vi "Save Library.vi"(8 "error in (no error)":errorcluster, 10 "Save Path (empty)":path, 11 "Library in":refnum<vi>) -> (0 "error out":errorcluster, 3 "Library out":refnum<vi>)   [LabVIEW 2019, in "gRPC Template Creation Utility.lvlib"]
uses:
  gRPC Template Creation Utility.lvlib
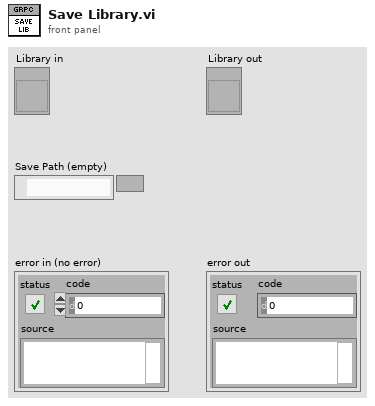
[diagram p1: front panel]
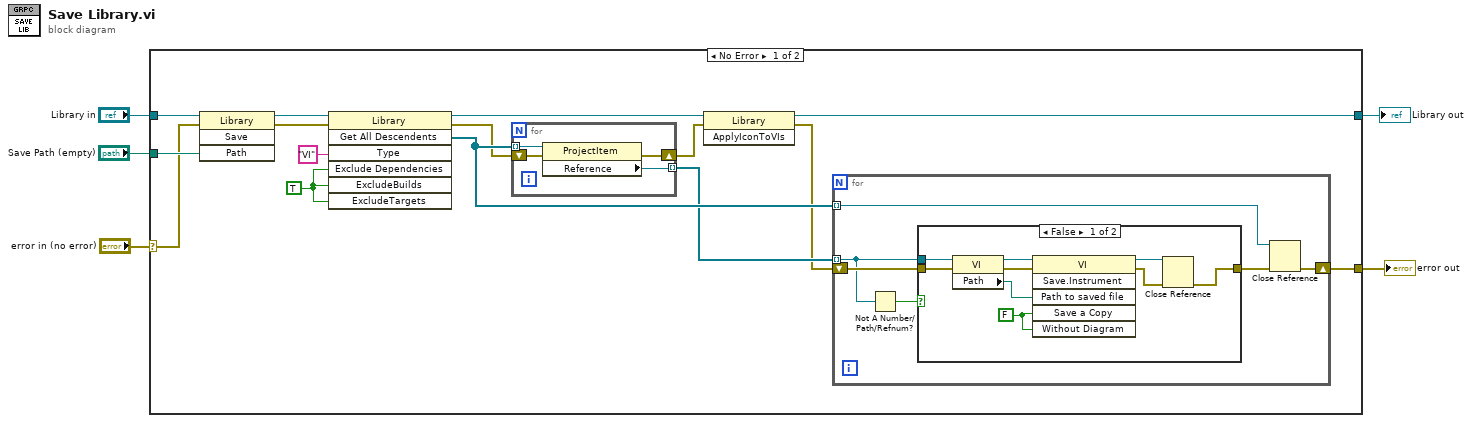
[diagram p0: block diagram]
diagram:
  n1 = case shown="No Error" "error in (no error)" {
    selector: "error in (no error)" -> [w18 w41]
    tunnel: [w15 w41] -> w5
    tunnel: [w8 w42] -> w4
    tunnel: "Library in" -> [w20 w42]
    tunnel: "Save Path (empty)" -> [w19 _]
    frame No Error {
      w16 = TRUE ("ExcludeBuilds")
      n2 = invoke class="Library" method="Save"(reference=w20, error in=w18, "Path"=w19) -> (reference out=w13:refnum<vi>, error out=w14:errorcluster)  [unwired: 1 in, 2 out]
      n3 = invoke class="Library" method="Get All Descendents"(reference=w13, error in=w14, "Type"="VI", "Exclude Dependencies"=w16, "ExcludeBuilds"=w16, "ExcludeTargets"=w16) -> (reference out=w9:refnum<vi>, error out=w11:errorcluster, "All Descendents"=w12:refnum<vi>[])  [unwired: 1 in, 4 out]
      n4 = for {
        tunnel: w12 -> [w24] mode=indexing
        shift-right: [w22] -> w10
        shift-left: w11 -> [w23]
        tunnel: [w21] -> w7 mode=indexing
        n5 = property class="ProjectItem"(reference=w24, error in=w23) -> (error out=w22:errorcluster, "Reference"=w21:refnum<vi>)  [unwired: 1 out]
      }
      n6 = invoke class="Library" method="ApplyIconToVIs"(reference=w9, error in=w10) -> (reference out=w8:refnum<vi>, error out=w6:errorcluster)  [unwired: 1 in, 1 out]
      n7 = for {
        tunnel: w12 -> [w25] mode=indexing
        shift-right: [w28] -> w15
        shift-left: w6 -> [w27]
        tunnel: w7 -> [w26] mode=indexing
        n8 = Not A Number/Path/Refnum?(number/path/refnum=w26) -> (NaN/Path/Refnum?=w30:bool)
        n9 = case shown="False" w30 {
          tunnel: [w33 w40] -> w29
          tunnel: w26 -> [w34 _]
          tunnel: w27 -> [w32 w40]
          frame False {
            w37 = FALSE ("Save a Copy")
            n10 = property class="VI"(reference=w34, error in=w32) -> (reference out=w39:refnum<vi>, error out=w38:errorcluster, "Path"=w31:path)
            n11 = invoke class="VI" method="Save.Instrument"(reference=w39, error in=w38, "Path to saved file"=w31, "Save a Copy"=w37, "Without Diagram"=w37) -> (reference out=w36:refnum<vi>, error out=w35:errorcluster)  [unwired: 1 in, 4 out]
            n12 = Close Reference(reference=w36, error in (no error)=w35) -> (error out=w33:errorcluster)
          }
          frame True {
          }
        }
        n13 = Close Reference(reference=w25, error in (no error)=w29) -> (error out=w28:errorcluster)
      }
    }
    frame Error {
    }
  }
  "error out" <- w5
  "Library out" <- w4
